vi "LVDeleteFile_Item_OnCommand.vi"(10 "Command ID":string, 11 "Object":T1) -> ()   [LabVIEW 2020]
uses:
  <resource>/Framework/Providers/API/ItemRef.ctl
panel:
  out "error out":errorcluster
  in  "error in":errorcluster
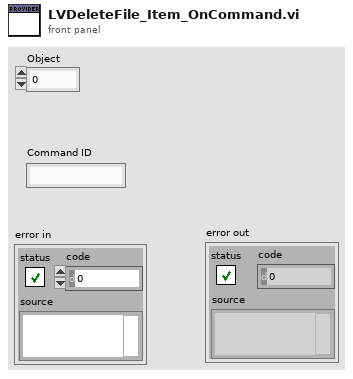
[diagram p1: front panel]
types:
  T1 = typedef "ItemRef.ctl" = u64
  T2 = typedef "ButtonDialogEnum.ctl" = enum16{"Left Button", "Middle Button", "Right Button", "Window Close"}
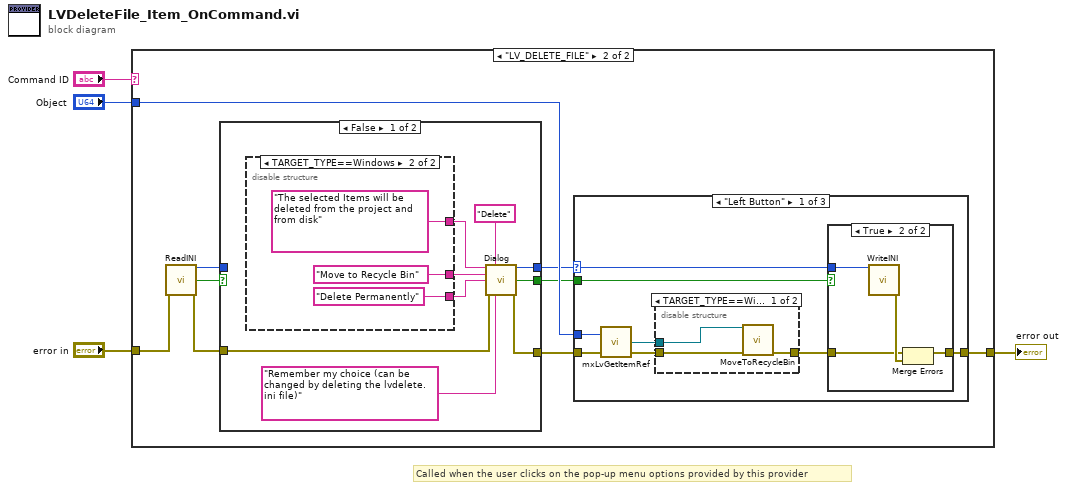
[diagram p0: block diagram]
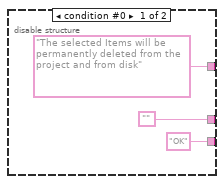
[diagram p3: hidden frame]
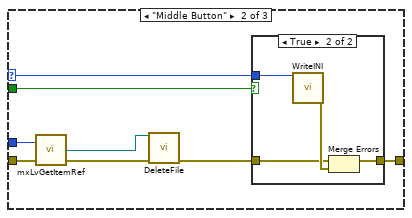
[diagram p7: hidden frame]
diagram:
  # "Called when the user clicks on the pop-up menu options provided by this provider"
  n1 = case shown="\"LV_DELETE_FILE\"" "Command ID" {
    tunnel: "error in" -> [w5 w9]
    tunnel: [w5 w14] -> w2
    tunnel: "Object" -> [_ w13]
    frame Default {
    }
    frame "LV_DELETE_FILE" {
      n2 = call "ReadINI.vi"("error in"=w9) -> ("Button"=w7:T2, "Found?"=w8:bool, "error out"=w10:errorcluster)  [unwired: 12 in]
      n3 = case shown="False" w8 {
        tunnel: [w22 w30] -> w12
        tunnel: [w18 w31] -> w11
        tunnel: w10 -> [w16 w31]
        tunnel: w7 -> [_ w30]
        tunnel: [w15 _] -> w6
        frame False {
          n4 = disable-structure shown="TARGET_TYPE==Windows" {
            disable-tunnel: ["The selected Items will be permanently deleted from the project and from disk" ("message") "The selected Items will be deleted from the project and from disk" ("message")] -> w23
            disable-tunnel: ["" "Move to Recycle Bin" ("message")] -> w21
            disable-tunnel: ["OK" ("message") "Delete Permanently" ("message")] -> w19
            frame condition #0 {
            }
            frame condition #1 (active) {
            }
          }
          n5 = call "Dialog.vi"("Message"=w23, "Title"="Delete" ("Window Title (\"\")"), "LeftButtonText(\"Yes\")"=w21, "MiddleButtonText(\"No\")"=w19, "error in"=w16, "CheckboxText"="Remember my choice (can be changed by deleting the lvdelete.ini file)") -> ("Enum"=w22:T2, "Checked?"=w15:bool, "error out"=w18:errorcluster)  [unwired: 7 in]
        }
        frame True {
        }
      }
      n6 = case shown="\"Left Button\"" w12 {
        selector: w12 -> [w32 w51 _]
        tunnel: w13 -> [w39 w56 _]
        tunnel: w11 -> [w38 w55 w62]
        tunnel: [w34 w49 w62] -> w14
        tunnel: w6 -> [w33 w52 _]
        frame "Left Button" {
          n7 = call <resource>:"mxLvGetItemRef.vi"("Item"=w39, "error in"=w38) -> ("Item Refnum"=w37:refnum<vi>, "error out"=w36:errorcluster)  [unwired: 1 out]
          n8 = disable-structure shown="TARGET_TYPE==Windows" {
            disable-tunnel: w37 -> [w47 _]
            disable-tunnel: w36 -> [w46 w48]
            disable-tunnel: [w45 w48] -> w35
            frame condition #0 (active) {
              n9 = call "MoveToRecycleBin.vi"("Item Refnum"=w47, "error in"=w46) -> ("error out"=w45:errorcluster)  [unwired: 13 in]
            }
            frame condition #1 {
            }
          }
          n10 = case shown="True" w33 {
            tunnel: w35 -> [w40 w41]
            tunnel: [w40 w42] -> w34
            tunnel: w32 -> [_ w43]
            frame False {
            }
            frame True {
              n11 = call "WriteINI.vi"("ButtonEnum"=w43) -> ("error out"=w44:errorcluster)  [unwired: 14 in]
              n12 = Merge Errors(w41, w44) -> (w42:errorcluster)
            }
          }
        }
        frame "Middle Button" {
          n13 = call <resource>:"mxLvGetItemRef.vi"("Item"=w56, "error in"=w55) -> ("Item Refnum"=w53:refnum<vi>, "error out"=w54:errorcluster)  [unwired: 1 out]
          n14 = call "DeleteFile.vi"("Item Refnum"=w53, "error in"=w54) -> ("error out"=w50:errorcluster)  [unwired: 13 in]
          n15 = case shown="True" w52 {
            tunnel: w50 -> [w57 w58]
            tunnel: [w57 w59] -> w49
            tunnel: w51 -> [_ w60]
            frame False {
            }
            frame True {
              n16 = call "WriteINI.vi"("ButtonEnum"=w60) -> ("error out"=w61:errorcluster)  [unwired: 14 in]
              n17 = Merge Errors(w58, w61) -> (w59:errorcluster)
            }
          }
        }
        frame Default {
        }
      }
    }
  }
  "error out" <- w2
